vi "Test_C_Receive.vi"() -> ()   [LabVIEW 2021]
uses:
  CANsub_C.lvlib
  common/CANsub_Common.lvlib
  common/Typedefs/REST_Phase.ctl
  typedefs/Test_RX_Stats.ctl
  common/Typedefs/CANsub_connection.ctl
  common/Typedefs/CANsub_Bit_Rates.ctl
panel:
  out "stats":T1 {"last data" format="%.0x"; "ids" format="%.0x"}
  out "error out":errorcluster
  out "closed by device":bool
  in  "CANsub_Bit_Rates":T2={"nominal bit rate"=500000, "nominal sample point"=80.0, "data bit rate"=2000000, "data sample point"=80.0}
  in  "CANsub_connection":T3={"host"="192.168.0.49", "channel"=2, "cert path"=path "/home/lvuser/cansub_root_cert.crt"}
  in  "run time (sec)":u32
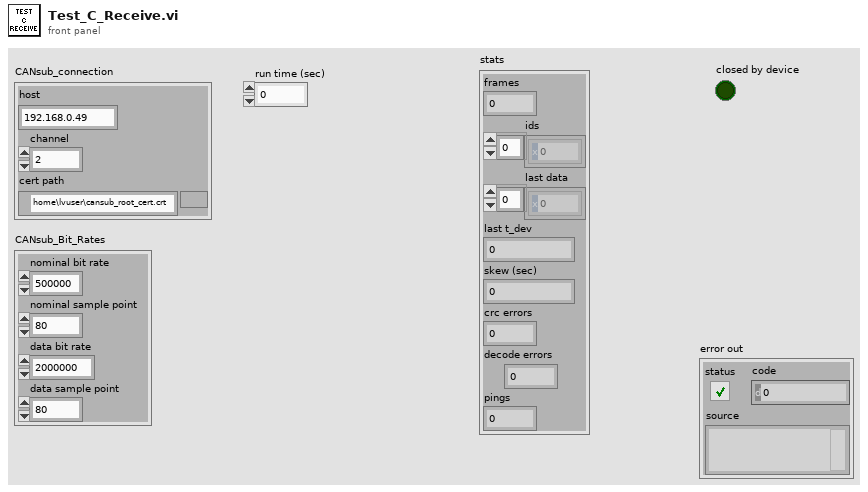
[diagram p1: front panel]
types:
  T1 = typedef "Test_RX_Stats.ctl" = cluster{"frames":i32, "ids":u32[], "last data":u8[], "last t_dev":dbl, "skew (sec)":dbl, "crc errors":u32, "decode errors":i32, "pings":i32}
  T2 = typedef "CANsub_Common.lvlib/CANsub_Bit_Rates.ctl" = cluster{"nominal bit rate":u32, "nominal sample point":dbl, "data bit rate":u32, "data sample point":dbl}
  T3 = typedef "CANsub_Common.lvlib/CANsub_connection.ctl" = cluster{"host":string, "channel":u8, "cert path":path}
  T4 = typedef "CANsub_Common.lvlib/REST_Phase.ctl" = enum16{"before_ws", "after_ws"}
  T5 = typedef "CANsub_Common.lvlib/Bit_Timing.ctl" = cluster{"brp":u16, "seg1":u16, "seg2":u16, "sjw":u16, "data brp":u16, "data seg1":u16, "data seg2":u16, "data sjw":u16}
  T6 = typedef "CANsub_C.lvlib/C_RX_Buffers.ctl" = cluster{"t_dev":dbl[], "ws":u8[], "id":u32[], "flags":u16[], "hdlc":u8[], "dlc":u8[], "data len":u8[], "data":u8[], "ping":u8[]}
  T7 = enum16{"Standard", "Buffered", "CRLF", "Immediate"}
  T8 = typedef "CANsub_C.lvlib/C_Decode_Result.ctl" = cluster{"n frames":i32, "peer close":bool, "ping len":i32, "crc errors":u32, "decode errors":i32}
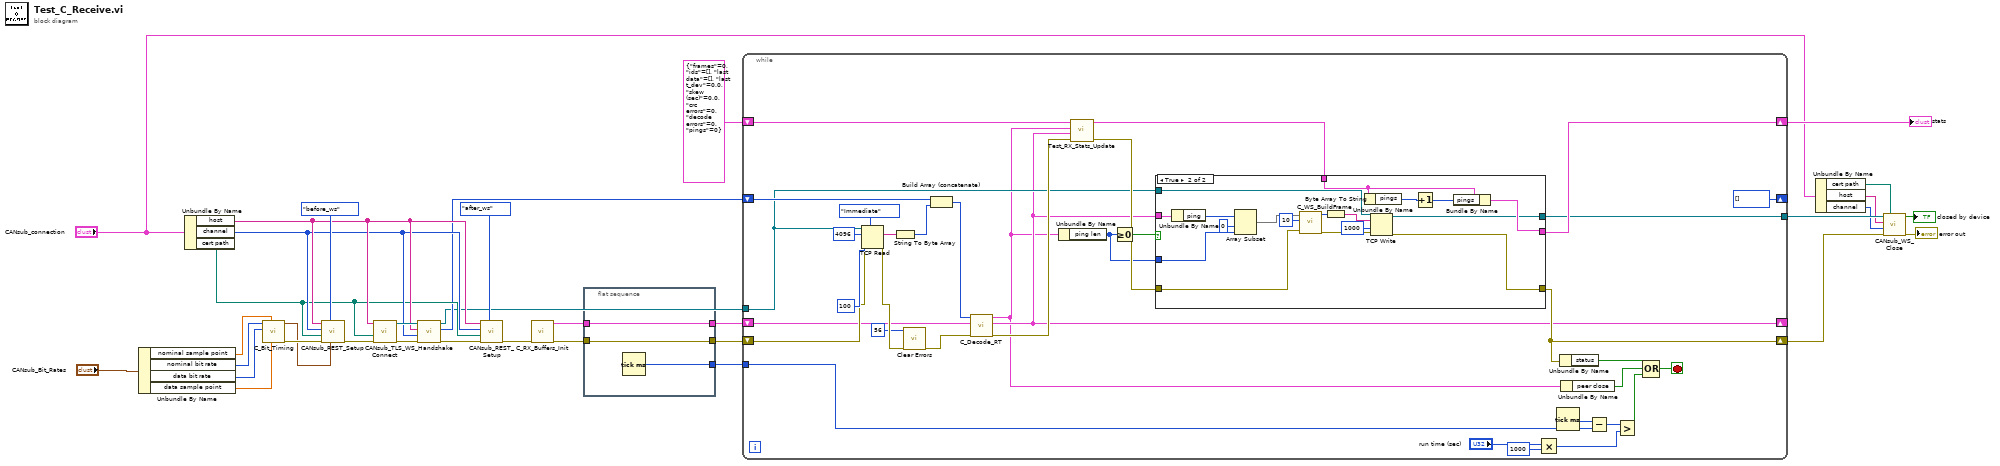
[diagram p0: block diagram]
diagram:
  n1 = Unbundle By Name("CANsub_Bit_Rates") -> ("nominal sample point"=w24:dbl, "nominal bit rate"=w27:u32, "data bit rate"=w26:u32, "data sample point"=w25:dbl)
  n2 = Unbundle By Name("CANsub_connection") -> ("host"=w20:string, "channel"=w19:u8, "cert path"=w18:path)
  n3 = call "C_Bit_Timing.vi"("data sample point"=w25, "nominal sample point"=w24, "data bit rate"=w26, "nominal bit rate"=w27) -> ("error out"=w33:errorcluster, "Bit_Timing"=w28:T5)  [unwired: 4 in, 2 out]
  n4 = call "CANsub_REST_Setup.vi"("bit timing"=w28, "phase"=REST_Phase."before_ws", "error in (no error)"=w33, "cert path"=w18, "channel"=w19, "host"=w20) -> ("error out"=w32:errorcluster)  [unwired: 4 in, 1 out]
  n5 = call "CANsub_TLS_Connect.vi"("error in (no error)"=w32, "cert path"=w18, "host"=w20) -> ("error out"=w31:errorcluster, "TLS connection"=w21:refnum<k5>)  [unwired: 6 in, 1 out]
  n6 = call "WS_Handshake.vi"("error in (no error)"=w31, "channel"=w19, "host"=w20, "TLS connection"=w21) -> ("error out"=w30:errorcluster, "leftover"=w13:u8[], "TLS connection out"=w11:refnum<k5>)  [unwired: 4 in, 1 out]
  n7 = call "CANsub_REST_Setup.vi"("phase"=REST_Phase."after_ws", "error in (no error)"=w30, "cert path"=w18, "channel"=w19, "host"=w20) -> ("error out"=w29:errorcluster)  [unwired: 5 in, 1 out]
  n8 = call "C_RX_Buffers_Init.vi"("error in (no error)"=w29) -> ("error out"=w17:errorcluster, "buffers"=w14:T6)  [unwired: 7 in, 2 out]
  n9 = flat-sequence {
    tunnel: [w37] -> w16
    tunnel: w17 -> [w37]
    tunnel: [w36] -> w9
    tunnel: [w35] -> w15
    tunnel: w14 -> [w35]
    frame #0 {
      n10 = Tick Count (ms)() -> (millisecond timer value=w36:u32)
    }
  }
  n11 = while {
    shift-right: [w56] -> w12
    shift-left: T1 {"frames"=0, "ids"=[], "last data"=[], "last t_dev"=0.0, "skew (sec)"=0.0, "crc errors"=0, "decode errors"=0, "pings"=0} ("stats") -> [w59]
    shift-right: [u8[] []] -> _
    shift-left: w13 -> [w65]
    shift-right: [w50] -> _
    shift-left: w15 -> [w62]
    shift-right: [w51] -> w3
    shift-left: w16 -> [w69]
    tunnel: w11 -> [w52]
    tunnel: w9 -> [w47]
    tunnel: [w38] -> w8
    stop <- w39 stop-if-true
    n12 = TCP Read(connection ID=w52, bytes to read=4096, error in (no error)=w69, 7:T7."Immediate" ("mode (standard)"), 9:100 ("timeout ms (25000)")) -> (data out=w66:string, error out=w68:errorcluster)  [unwired: 1 out]
    n13 = String To Byte Array(string=w66) -> (unsigned byte array=w64:u8[])
    n14 = call <vilib>:"Clear Errors.vi"("error in (no error)"=w68, "specific error code to clear (0: all)"=56) -> ("error out"=w60:errorcluster)  [unwired: 4 in, 1 out]
    n15 = Build Array (concatenate)(w65, w64) -> (w61:u8[])
    n16 = call "C_Decode_RT.vi"("error in (no error)"=w60, "buffers in"=w62, "bytes in"=w61) -> ("error out"=w55:errorcluster, "buffers out"=w50:T6, "result"=w49:T8)  [unwired: 6 in]
    n17 = Unbundle By Name(w49) -> ("ping len"=w53:i32)
    n18 = call "Test_RX_Stats_Update.vi"("error in (no error)"=w55, "buffers in"=w50, "result"=w49, "stats in"=w59) -> ("error out"=w54:errorcluster, "stats out"=w57:T1)  [unwired: 6 in]
    n19 = Greater Or Equal To 0?(x=w53) -> (x >= 0?=w58:bool)
    n20 = case shown="True" w58 {
      tunnel: w57 -> [w74 w81]
      tunnel: [w74 w80] -> w56
      tunnel: w54 -> [w75 w88]
      tunnel: [w75 w82] -> w51
      tunnel: w50 -> [_ w93]
      tunnel: w53 -> [_ w90]
      tunnel: w52 -> [w73 w86]
      tunnel: [w73 w76] -> w38
      frame False {
      }
      frame True {
        n21 = Unbundle By Name(w93) -> ("ping"=w92:u8[])
        n22 = Array Subset(array=w92, index=0, length=w90) -> (w77:u8[])
        n23 = call "C_WS_BuildFrame.vi"("error in (no error)"=w88, "opcode"=u8 10, "payload"=w77) -> ("error out"=w83:errorcluster, "frame"=w87:u8[])  [unwired: 7 in]
        n24 = Byte Array To String(unsigned byte array=w87) -> (string=w85:string)
        n25 = Unbundle By Name(w81) -> ("pings"=w79:i32)
        n26 = TCP Write(connection ID=w86, data in=w85, error in (no error)=w83, 9:1000 ("timeout ms (25000)")) -> (connection ID out=w76:refnum<k5>, error out=w82:errorcluster)  [unwired: 1 out]
        n27 = Increment(x=w79) -> (x+1=w78:i32)
        n28 = Bundle By Name(cluster=w81, "pings"=w78) -> (w80:T1)
      }
    }
    n29 = Multiply(x="run time (sec)", y=u32 1000) -> (x*y=w44:u32)
    n30 = Tick Count (ms)() -> (millisecond timer value=w48:u32)
    n31 = Unbundle By Name(w51) -> ("status"=w42:bool)
    n32 = Unbundle By Name(w49) -> ("peer close"=w41:bool)
    n33 = Subtract(x=w48, y=w47) -> (x-y=w43:u32)
    n34 = Greater?(x=w43, y=w44) -> (0:w40:bool)
    n35 = Compound Arithmetic op=OR(w42, w41, w40) -> (w39:bool)
  }
  "stats" <- w12
  n36 = Unbundle By Name("CANsub_connection") -> ("cert path"=w6:path, "host"=w5:string, "channel"=w4:u8)
  n37 = call "CANsub_WS_Close.vi"("cert path"=w6, "error in (no error)"=w3, "channel"=w4, "host"=w5, "TLS Connection"=w8) -> ("error out"=→"error out":errorcluster, "closed by device"=→"closed by device":bool)  [unwired: 5 in]
